vi "Aquring Samples.vi"(8 "error in":errorcluster, 9 "rate":dbl=25000.0, 10 "number of samples":i32=25000) -> (0 "error out":errorcluster, 3 "task out":refnum<k21>)   [LabVIEW 2020]
uses:
  <vilib>/DAQmx/create/channels.llb/DAQmx Create Channel (AI-Force-Bridge-Two-Point-Linear).vi
  <vilib>/DAQmx/configure/timing.llb/DAQmx Timing (Sample Clock).vi
  <resource>/objmgr/daqmx.rc
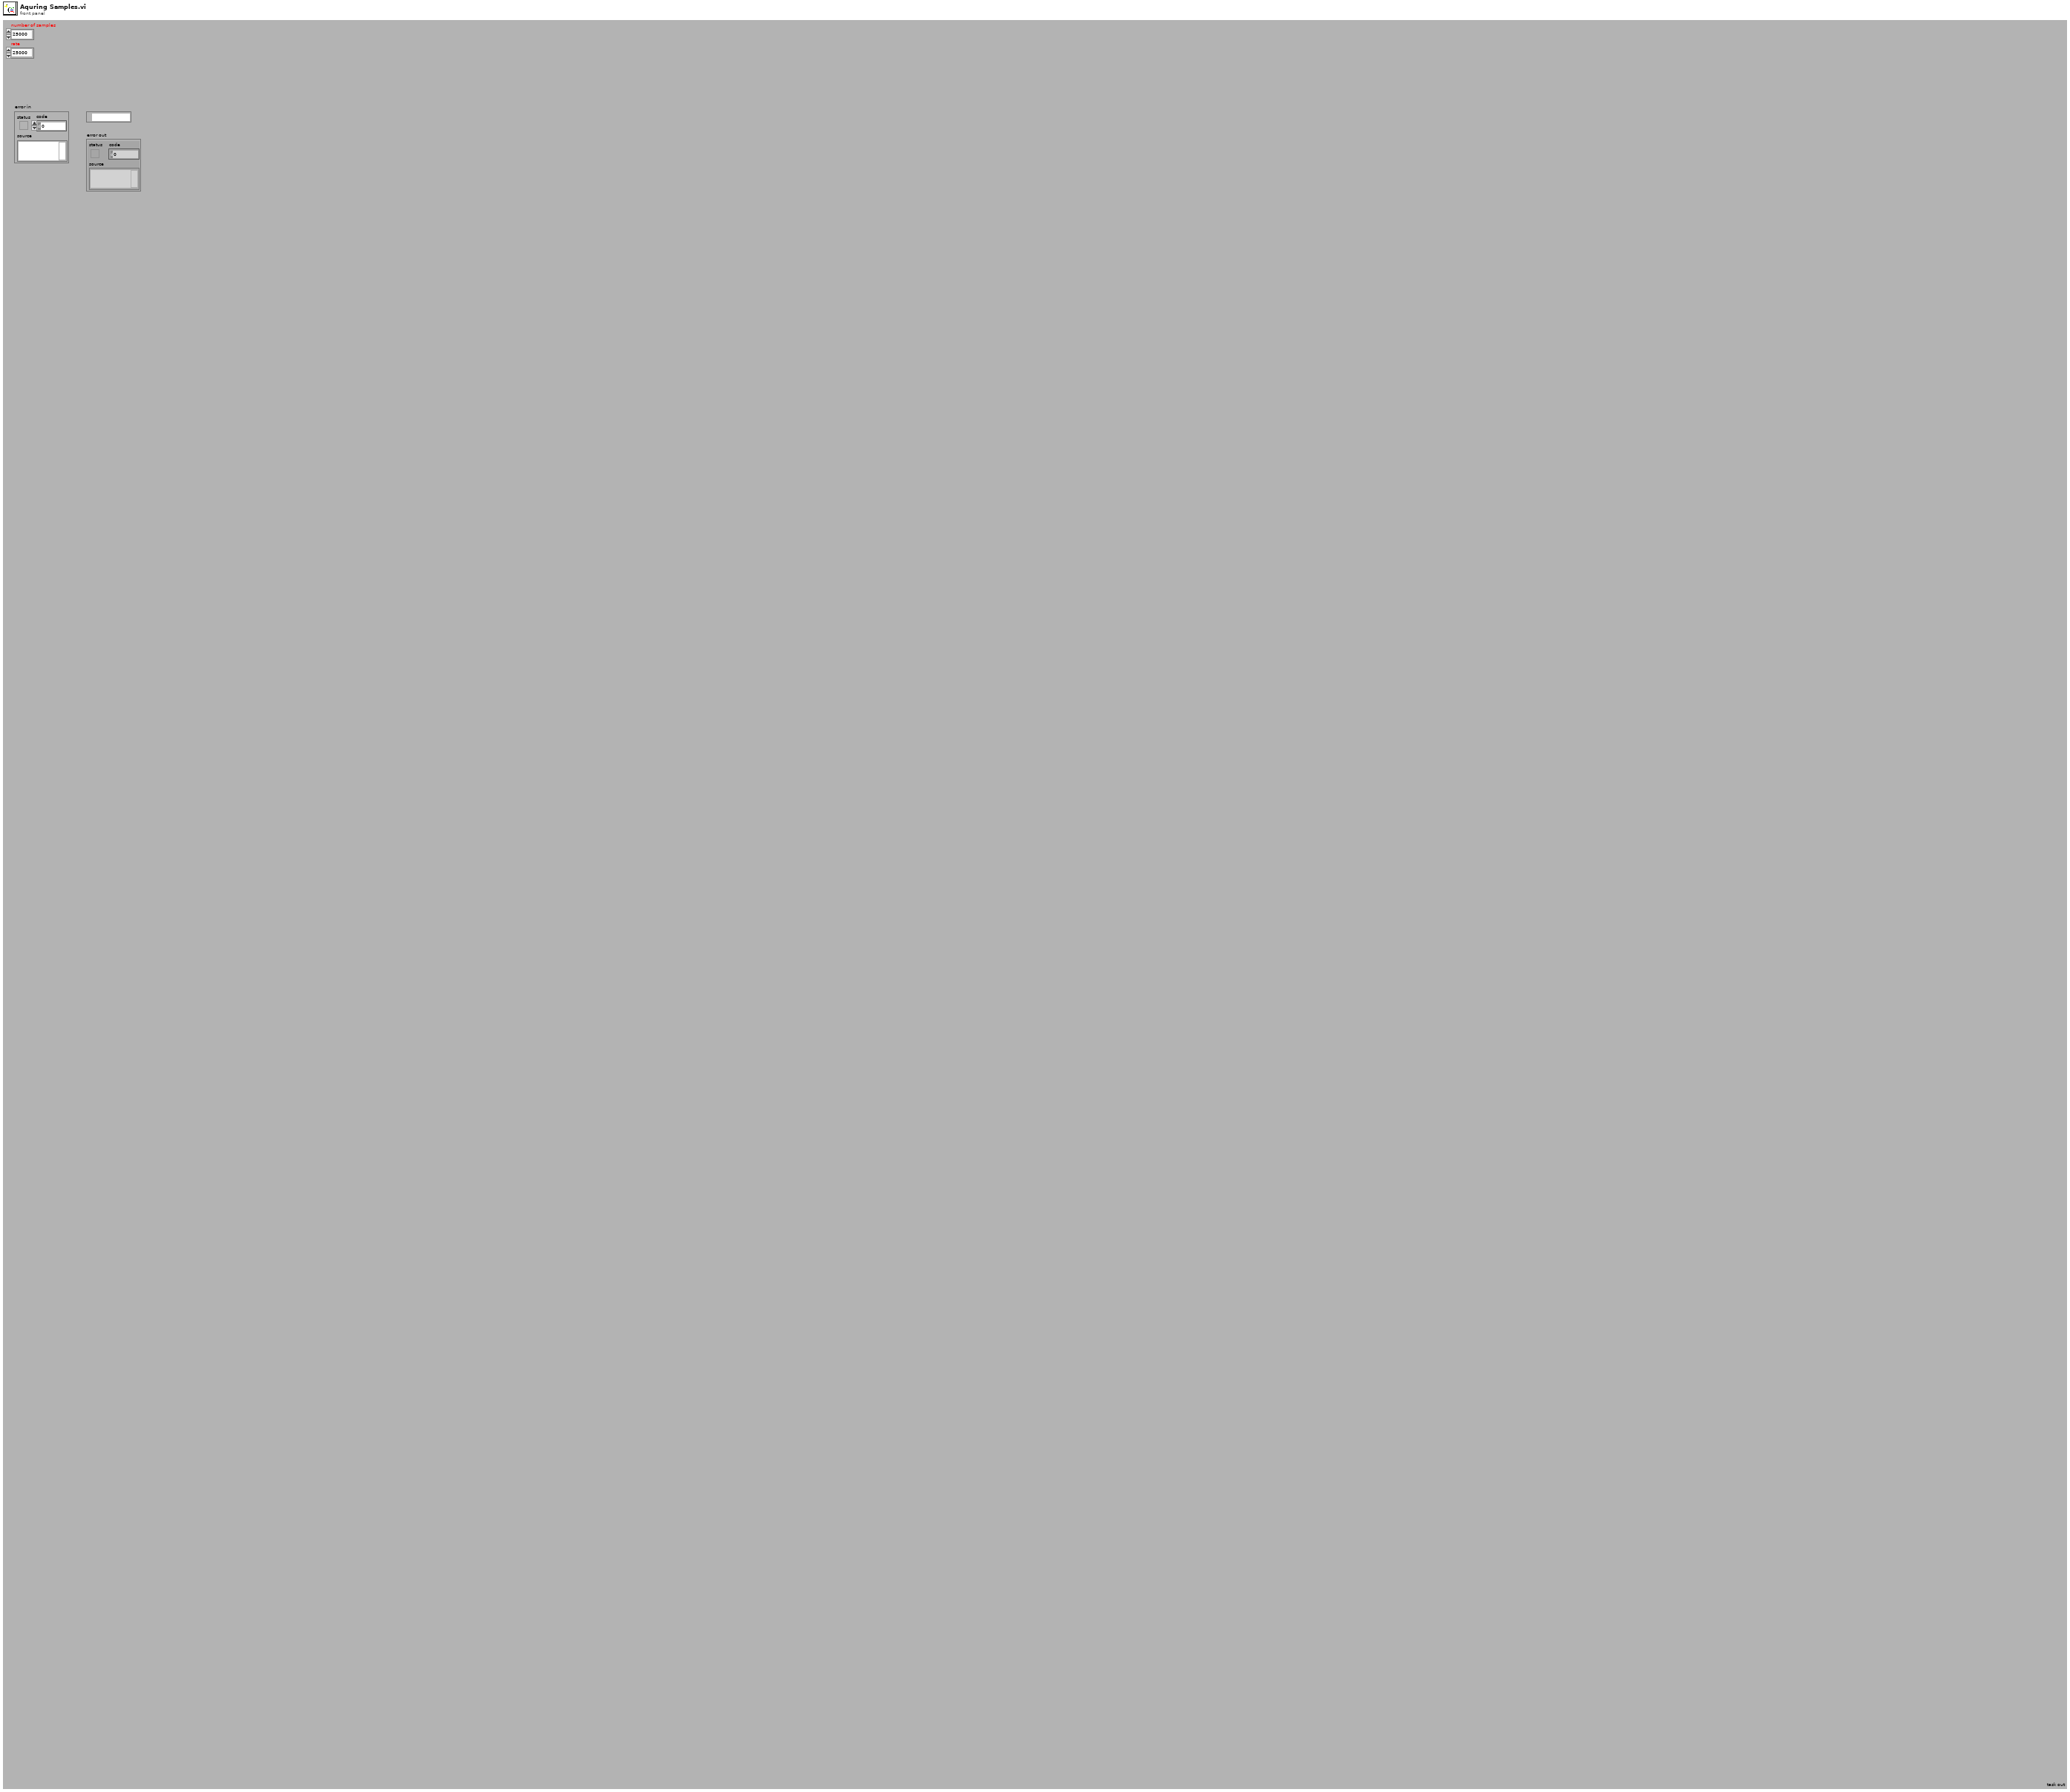
[diagram p1: front panel]
types:
  T1 = cluster{"bridge configuration":i32, "voltage excitation source":i32, "voltage excitation value":dbl, "nominal bridge resistance":dbl}
  T2 = cluster{"first electrical value":dbl, "second electrical value":dbl, "electrical units":i32, "first physical value":dbl, "second physical value":dbl, "physical units":i32}
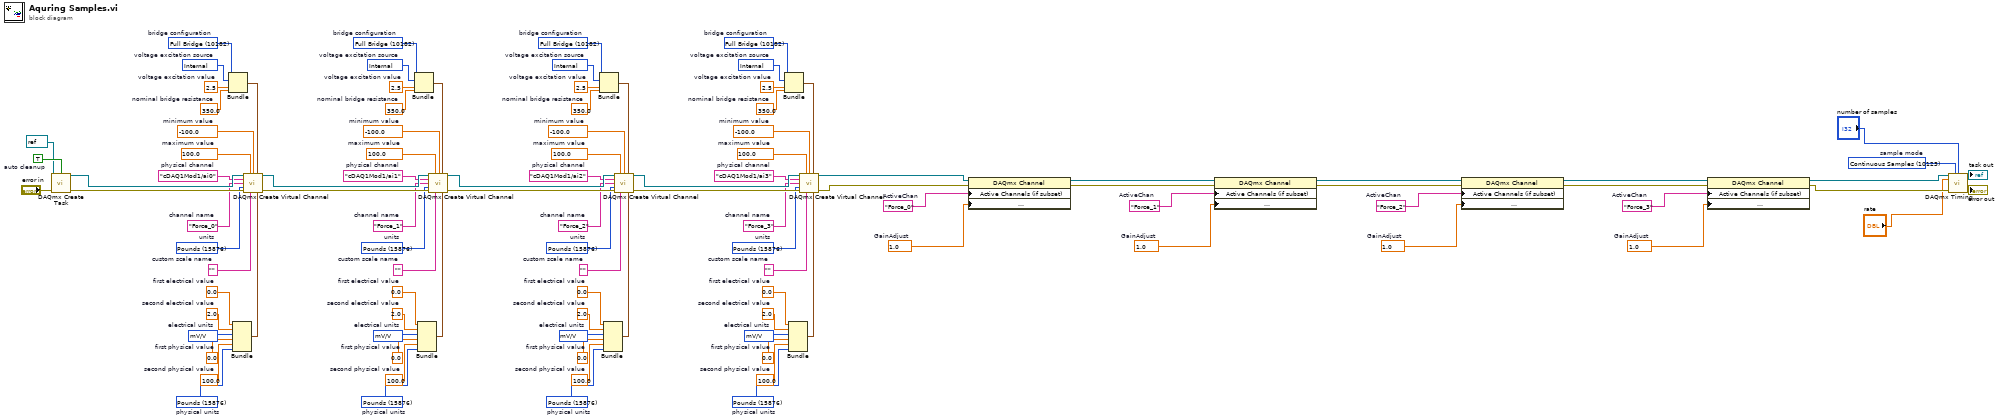
[diagram p0: block diagram]
diagram:
  w4 = 10123 items=["Finite Samples"=10178, "Continuous Samples"=10123, "Hardware Timed Single Point"=12522]  # sample mode
  w8 = 1.0  # GainAdjust
  w11 = "Force_3"  # ActiveChan
  w12 = 1.0  # GainAdjust
  w15 = "Force_2"  # ActiveChan
  w16 = 1.0  # GainAdjust
  w19 = "Force_1"  # ActiveChan
  w20 = 1.0  # GainAdjust
  w23 = "Force_0"  # ActiveChan
  w24 = 15876 items=["Newtons"=15875, "Pounds"=15876, "kgf"=15877]  # physical units
  w30 = 0.0  # first electrical value
  w29 = 2.0  # second electrical value
  w28 = 15897 items=["V/V"=15896, "mV/V"=15897]  # electrical units
  w27 = 0.0  # first physical value
  w26 = 100.0  # second physical value
  w32 = 350.0  # nominal bridge resistance
  w33 = 2.5  # voltage excitation value
  w34 = 10200 items=["Internal"=10200, "External"=10167]  # voltage excitation source
  w35 = 10182 items=["Full Bridge"=10182, "Half Bridge"=10187, "Quarter Bridge"=10270]  # bridge configuration
  w36 = 15876 items=["Newtons"=15875, "Pounds"=15876, "kgf"=15877, "From Custom Scale"=10065]  # units
  w37 = "Force_3"  # channel name
  w39 = ""  # custom scale name
  w40 = -100.0  # minimum value
  w41 = 100.0  # maximum value
  w42 = "cDAQ1Mod1/ai3"  # physical channel
  w44 = 15876 items=["Newtons"=15875, "Pounds"=15876, "kgf"=15877]  # physical units
  w50 = 0.0  # first electrical value
  w49 = 2.0  # second electrical value
  w48 = 15897 items=["V/V"=15896, "mV/V"=15897]  # electrical units
  w47 = 0.0  # first physical value
  w46 = 100.0  # second physical value
  w52 = 350.0  # nominal bridge resistance
  w53 = 2.5  # voltage excitation value
  w54 = 10200 items=["Internal"=10200, "External"=10167]  # voltage excitation source
  w55 = 10182 items=["Full Bridge"=10182, "Half Bridge"=10187, "Quarter Bridge"=10270]  # bridge configuration
  w56 = 15876 items=["Newtons"=15875, "Pounds"=15876, "kgf"=15877, "From Custom Scale"=10065]  # units
  w57 = "Force_2"  # channel name
  w59 = ""  # custom scale name
  w60 = -100.0  # minimum value
  w61 = 100.0  # maximum value
  w62 = "cDAQ1Mod1/ai2"  # physical channel
  w64 = 15876 items=["Newtons"=15875, "Pounds"=15876, "kgf"=15877]  # physical units
  w70 = 0.0  # first electrical value
  w69 = 2.0  # second electrical value
  w68 = 15897 items=["V/V"=15896, "mV/V"=15897]  # electrical units
  w67 = 0.0  # first physical value
  w66 = 100.0  # second physical value
  w72 = 350.0  # nominal bridge resistance
  w73 = 2.5  # voltage excitation value
  w74 = 10200 items=["Internal"=10200, "External"=10167]  # voltage excitation source
  w75 = 10182 items=["Full Bridge"=10182, "Half Bridge"=10187, "Quarter Bridge"=10270]  # bridge configuration
  w76 = 15876 items=["Newtons"=15875, "Pounds"=15876, "kgf"=15877, "From Custom Scale"=10065]  # units
  w77 = "Force_1"  # channel name
  w79 = ""  # custom scale name
  w80 = -100.0  # minimum value
  w81 = 100.0  # maximum value
  w82 = "cDAQ1Mod1/ai1"  # physical channel
  w84 = 15876 items=["Newtons"=15875, "Pounds"=15876, "kgf"=15877]  # physical units
  w90 = 0.0  # first electrical value
  w89 = 2.0  # second electrical value
  w88 = 15897 items=["V/V"=15896, "mV/V"=15897]  # electrical units
  w87 = 0.0  # first physical value
  w86 = 100.0  # second physical value
  w92 = 350.0  # nominal bridge resistance
  w93 = 2.5  # voltage excitation value
  w94 = 10200 items=["Internal"=10200, "External"=10167]  # voltage excitation source
  w95 = 10182 items=["Full Bridge"=10182, "Half Bridge"=10187, "Quarter Bridge"=10270]  # bridge configuration
  w96 = 15876 items=["Newtons"=15875, "Pounds"=15876, "kgf"=15877, "From Custom Scale"=10065]  # units
  w97 = "Force_0"  # channel name
  w99 = ""  # custom scale name
  w100 = -100.0  # minimum value
  w101 = 100.0  # maximum value
  w102 = "cDAQ1Mod1/ai0"  # physical channel
  w104 = TRUE  # auto cleanup
  n1 = call <vilib>:"DAQmx Create Task.vi"("auto cleanup"=w104, "task to copy"=refnum<k21> refnum, "error in"="error in") -> ("task out"=w103:refnum<k21>, "error out"=w105:errorcluster)  [unwired: 11 in]
  n2 = Bundle("bridge configuration"=w95, "voltage excitation source"=w94, "voltage excitation value"=w93, "nominal bridge resistance"=w92) -> (w91:T1)  [unwired: 1 in]
  n3 = Bundle("first electrical value"=w90, "second electrical value"=w89, "electrical units"=w88, "first physical value"=w87, "second physical value"=w86, "physical units"=w84) -> (w85:T2)  [unwired: 1 in]
  n4 = call-poly <vilib>:"DAQmx Create Virtual Channel.vi"("task in"=w103, "maximum value"=w101, "minimum value"=w100, "bridge information"=w91, "physical channels"=w102, "name to assign"=w97, "units"=w96, "error in"=w105, "custom scale name"=w99, "scaling information"=w85) -> ("task out"=w83:refnum<k21>, "error out"=w98:errorcluster)  [unwired: 4 in]
  n5 = Bundle("bridge configuration"=w75, "voltage excitation source"=w74, "voltage excitation value"=w73, "nominal bridge resistance"=w72) -> (w71:T1)  [unwired: 1 in]
  n6 = Bundle("first electrical value"=w70, "second electrical value"=w69, "electrical units"=w68, "first physical value"=w67, "second physical value"=w66, "physical units"=w64) -> (w65:T2)  [unwired: 1 in]
  n7 = call-poly <vilib>:"DAQmx Create Virtual Channel.vi"("task in"=w83, "maximum value"=w81, "minimum value"=w80, "bridge information"=w71, "physical channels"=w82, "name to assign"=w77, "units"=w76, "error in"=w98, "custom scale name"=w79, "scaling information"=w65) -> ("task out"=w63:refnum<k21>, "error out"=w78:errorcluster)  [unwired: 4 in]
  n8 = Bundle("bridge configuration"=w55, "voltage excitation source"=w54, "voltage excitation value"=w53, "nominal bridge resistance"=w52) -> (w51:T1)  [unwired: 1 in]
  n9 = Bundle("first electrical value"=w50, "second electrical value"=w49, "electrical units"=w48, "first physical value"=w47, "second physical value"=w46, "physical units"=w44) -> (w45:T2)  [unwired: 1 in]
  n10 = call-poly <vilib>:"DAQmx Create Virtual Channel.vi"("task in"=w63, "maximum value"=w61, "minimum value"=w60, "bridge information"=w51, "physical channels"=w62, "name to assign"=w57, "units"=w56, "error in"=w78, "custom scale name"=w59, "scaling information"=w45) -> ("task out"=w43:refnum<k21>, "error out"=w58:errorcluster)  [unwired: 4 in]
  n11 = Bundle("bridge configuration"=w35, "voltage excitation source"=w34, "voltage excitation value"=w33, "nominal bridge resistance"=w32) -> (w31:T1)  [unwired: 1 in]
  n12 = Bundle("first electrical value"=w30, "second electrical value"=w29, "electrical units"=w28, "first physical value"=w27, "second physical value"=w26, "physical units"=w24) -> (w25:T2)  [unwired: 1 in]
  n13 = call-poly <vilib>:"DAQmx Create Virtual Channel.vi"("task in"=w43, "maximum value"=w41, "minimum value"=w40, "bridge information"=w31, "physical channels"=w42, "name to assign"=w37, "units"=w36, "error in"=w58, "custom scale name"=w39, "scaling information"=w25) -> ("task out"=w22:refnum<k21>, "error out"=w38:errorcluster)  [unwired: 4 in]
  n14 = property class="DAQmx Channel"(reference=w22, error in=w38, "Active Channels (if subset)"=w23, "Analog Input:General Properties:Signal Conditioning:Bridge:Shunt Cal:Gain Adjustment"=w20) -> (reference out=w18:refnum<k21>, error out=w21:errorcluster)
  n15 = property class="DAQmx Channel"(reference=w18, error in=w21, "Active Channels (if subset)"=w19, "Analog Input:General Properties:Signal Conditioning:Bridge:Shunt Cal:Gain Adjustment"=w16) -> (reference out=w14:refnum<k21>, error out=w17:errorcluster)
  n16 = property class="DAQmx Channel"(reference=w14, error in=w17, "Active Channels (if subset)"=w15, "Analog Input:General Properties:Signal Conditioning:Bridge:Shunt Cal:Gain Adjustment"=w12) -> (reference out=w10:refnum<k21>, error out=w13:errorcluster)
  n17 = property class="DAQmx Channel"(reference=w10, error in=w13, "Active Channels (if subset)"=w11, "Analog Input:General Properties:Signal Conditioning:Bridge:Shunt Cal:Gain Adjustment"=w8) -> (reference out=w5:refnum<k21>, error out=w9:errorcluster)
  n18 = call-poly <vilib>:"DAQmx Timing.vi"("task/channels in"=w5, "sample mode"=w4, "samples per channel"="number of samples", "rate"="rate", "error in"=w9) -> ("task out"=→"task out":refnum<k21>, "error out"=→"error out":errorcluster)  [unwired: 9 in]
